vi "RemoteVI Capture Panel.vi"(8 "error in":errorcluster, 11 "VI":refnum<vi>) -> (0 "error out":errorcluster, 1 "height":i32, 2 "width":i32, 3 "pixmap":u32[][](array[numeric]))   [LabVIEW 2020, in "RemoteVI.lvlib"]
doc: "Grabs the visible area of the front panel of VI as a 24-bit image (FP.Get Image, visible area only, image depth 24) and unflattens it to a 2D U32 pixmap [row, column] with one 0x00RRGGBB value per pixel. width and height are read from the pixmap's dimensions. The panel must be open for the image to show the panel's content. On an error (including an error at error in) pixmap is empty, width and height are 0 and the error is returned in error out."
uses:
  RemoteVI.lvlib
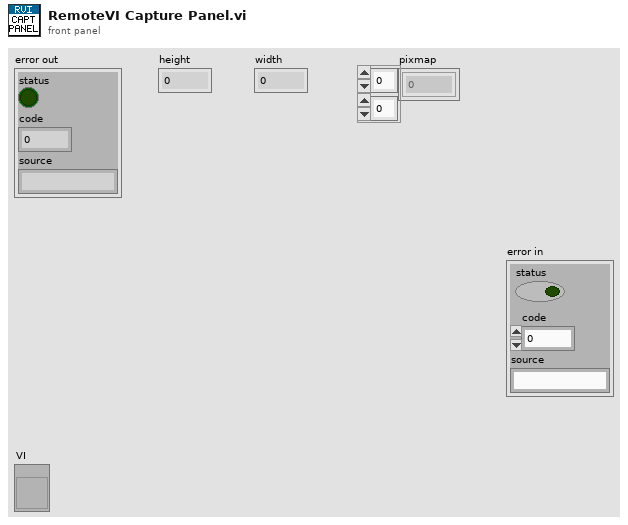
[diagram p1: front panel]
types:
  T1 = typedef "imagedata.ctl" = cluster{"image type":i32, "image depth":i32, "image":u8[], "mask":u8[], "colors":u32[], "Rectangle":cluster{"left":i16, "top":i16, "right":i16, "bottom":i16}}
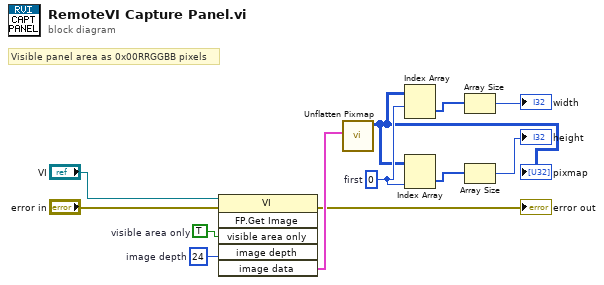
[diagram p0: block diagram]
diagram:
  w9 = 0  # first
  w8 = 24  # image depth
  w7 = TRUE  # visible area only
  # "Visible panel area as 0x00RRGGBB pixels"
  n1 = invoke class="VI" method="FP.Get Image"(reference="VI", error in="error in", "visible area only"=w7, "image depth"=w8) -> (error out=→"error out":errorcluster, "image data"=w10:T1)  [unwired: 2 in, 4 out]
  n2 = call <vilib>:"Unflatten Pixmap.vi"("image data"=w10) -> ("24-bit pixmap"=w3:u32[][])  [unwired: 4 in, 6 out]
  "pixmap" <- w3
  n3 = Index Array(array=w3, index (row)=w9) -> (element=w11:u32[])  [unwired: 1 in]
  n4 = Index Array(array=w3, index (col)=w9) -> (element=w12:u32[])  [unwired: 1 in]
  n5 = Array Size(array=w11) -> (size(s)=→"width":i32)
  n6 = Array Size(array=w12) -> (size(s)=→"height":i32)
